vi "Data Serie to Waveform.vi"(11 "Data Serie A":T1) -> (3 "Waveform":waveform(dbl))   [LabVIEW 2020, in "Data Viewer.lvlib" / "Data Viewer.lvclass"]
uses:
  Data Viewer.lvclass
  Data Serie--cluster.ctl
  Data Viewer.lvlib
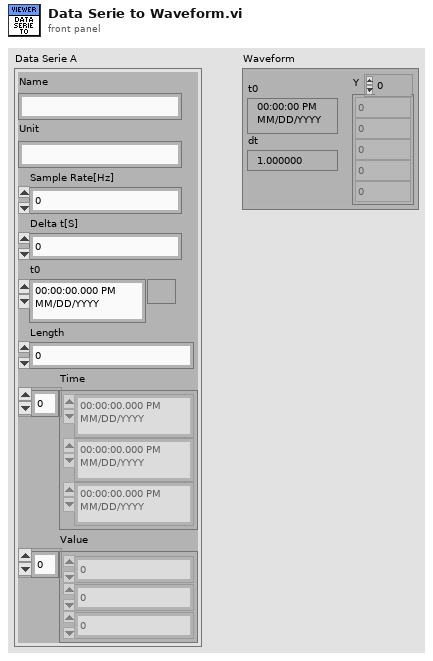
[diagram p1: front panel]
types:
  T1 = typedef "Data Viewer.lvlib/Data Serie--cluster.ctl" = cluster{"Name":string, "Unit":string, "Sample Rate[Hz]":dbl, "Delta t[S]":dbl, "t0":timestamp, "Length":i32, "Time":timestamp[], "Value":dbl[]}
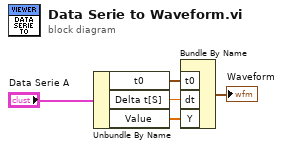
[diagram p0: block diagram]
diagram:
  n1 = Unbundle By Name("Data Serie A") -> ("t0"=w2:timestamp, "Delta t[S]"=w3:dbl, "Value"=w4:dbl[])
  n2 = Bundle By Name("t0"=w2, "dt"=w3, "Y"=w4) -> (→"Waveform":waveform(dbl))  [unwired: 1 in]
